vi "RemoteVI Send Frame.vi"(0 "Client":T1, 5 "pixmap":u32[][](array[numeric]), 7 "width":i32, 9 "height":i32, 11 "error in":errorcluster) -> (4 "Client out":T1, 6 "sent?":bool, 15 "error out":errorcluster)   [LabVIEW 2020, in "RemoteVI.lvlib"]
doc: "Sends one FRAME to one client if flow control allows (docs\\protocol.md sections 3.1 and 5). Nothing happens when the client is closed or already has 2 unacknowledged frames (seq - acked >= 2), or when RemoteVI Dirty Rects.vi finds no change against the pixmap this client was last sent. Otherwise every dirty rect is encoded with RemoteVI Encode Rect PNG.vi, the frame is built with RemoteVI Frame Encode.vi (seq + 1, width, height), wrapped in a binary WebSocket frame and written with TCP Write (2 s timeout). On success seq is incremented, last sent becomes pixmap and sent? is TRUE; a write error sets closed instead. error out carries PNG encoding errors."
uses:
  RemoteVI.lvlib
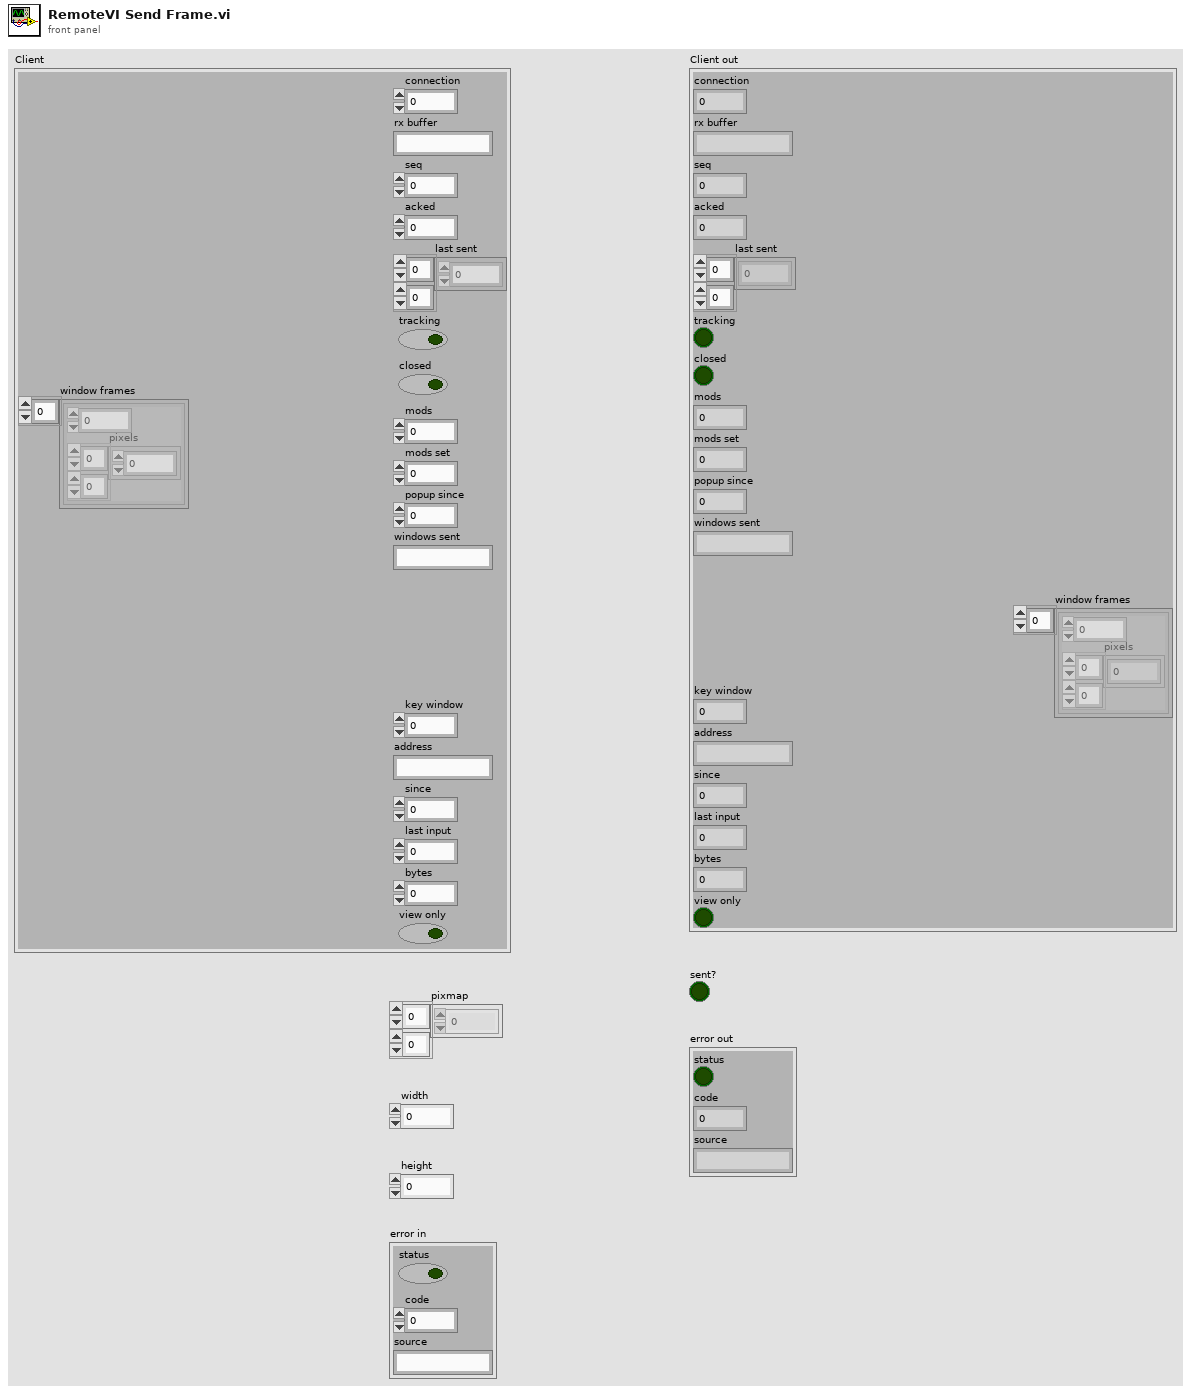
[diagram p1: front panel]
types:
  T1 = cluster{"connection":u32, "rx buffer":string, "seq":u32, "acked":u32, "last sent":u32[][], "tracking":bool, "closed":bool, "mods":u8, "mods set":u8, "popup since":u32, "windows sent":string, "window frames":cluster{"id":u64, "pixels":u32[][]}[], "key window":u64, "address":string, "since":dbl, "last input":dbl, "bytes":dbl, "view only":bool}
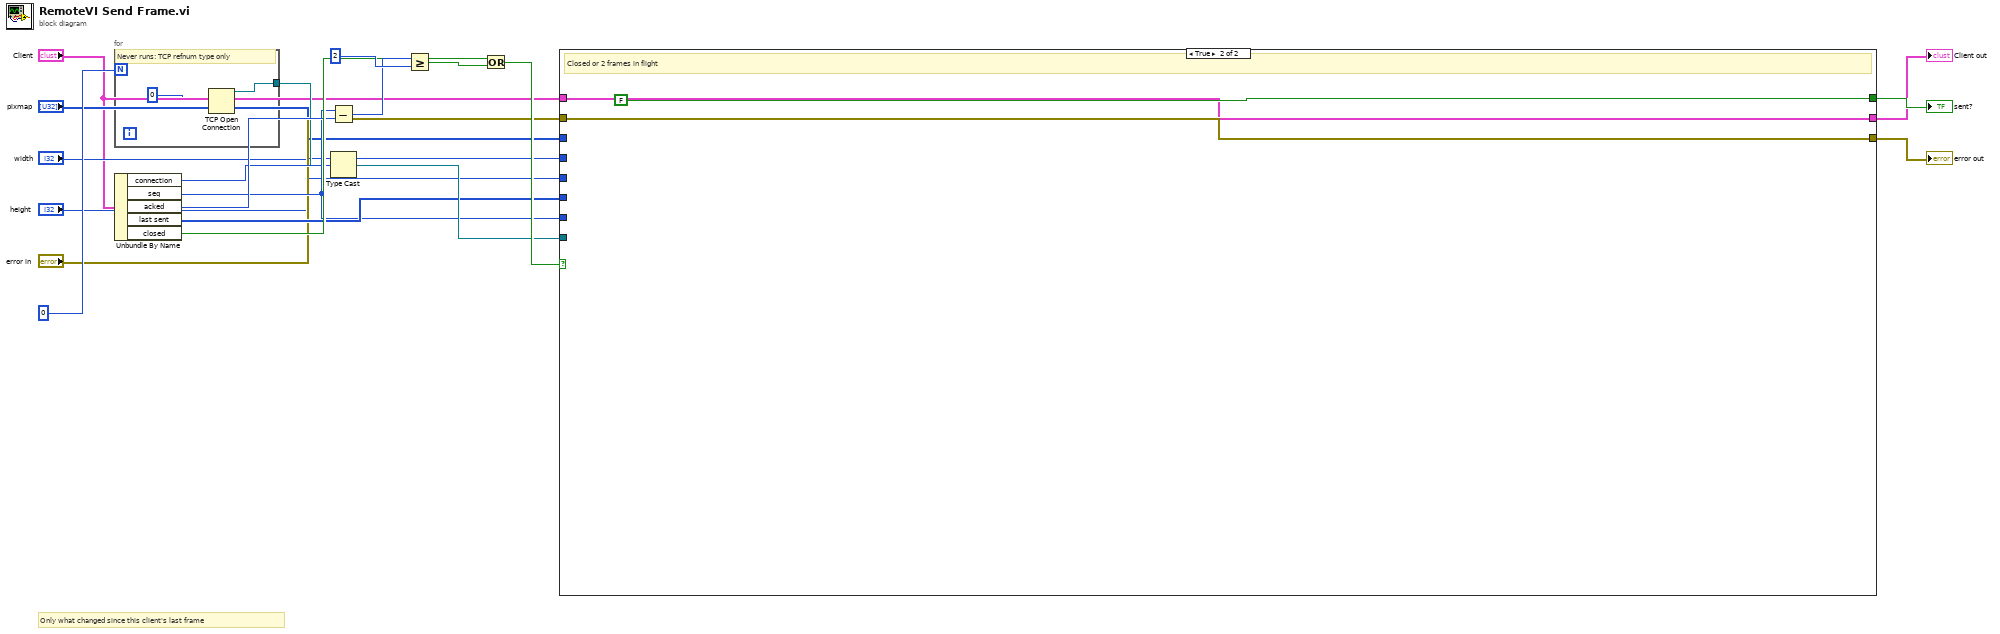
[diagram p0: block diagram]
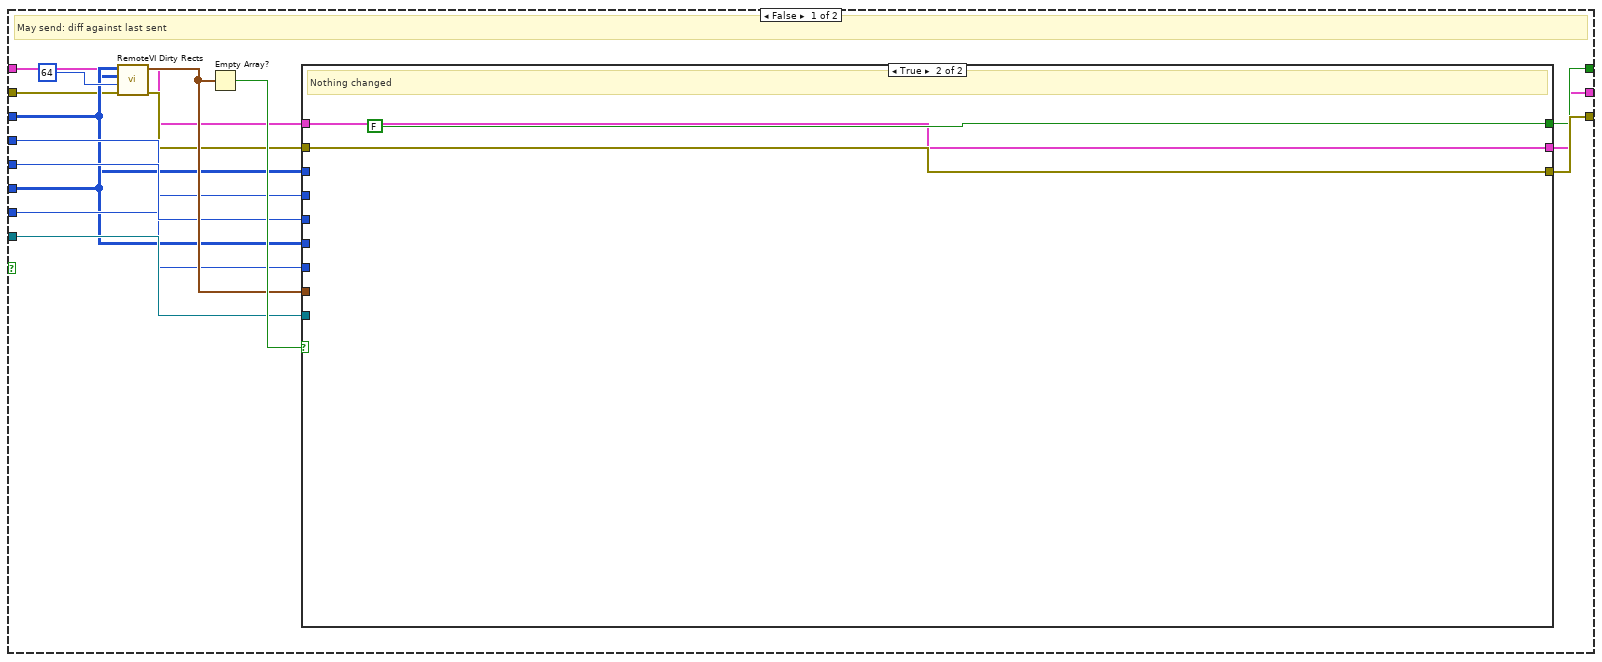
[diagram p2: hidden frame]
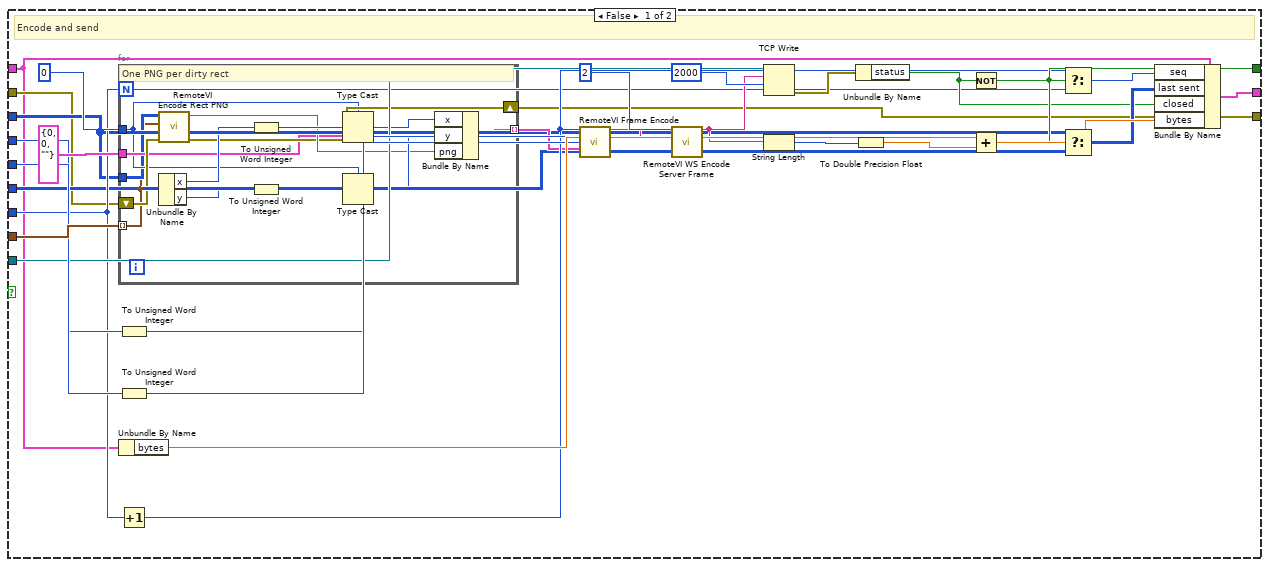
[diagram p3: hidden frame]
diagram:
  # "Only what changed since this client's last frame"
  n1 = for {
    N: 0 -> [_]
    tunnel: [w22] -> w7
    # "Never runs: TCP refnum type only"
    n2 = TCP Open Connection(remote port or service name=u16 0) -> (connection ID=w22:refnum<k5>)  [unwired: 4 in, 1 out]
  }
  n3 = Unbundle By Name("Client") -> ("connection"=w8:u32, "seq"=w9:u32, "acked"=w10:u32, "last sent"=w11:u32[][], "closed"=w12:bool)
  n4 = Subtract(x=w9, y=w10) -> (x-y=w14:u32)
  n5 = Type Cast(type=w7, x=w8) -> (*(type *) &x=w13:refnum<k5>)
  n6 = Greater Or Equal?(x=w14, y=u32 2) -> (x >= y?=w16:bool)
  n7 = Or(x=w12, y=w16) -> (x .or. y?=w17:bool)
  n8 = case shown="True" w17 {
    tunnel: "Client" -> [w23 w84]
    tunnel: "error in" -> [w24 w85]
    tunnel: "pixmap" -> [w25 _]
    tunnel: "width" -> [w29 _]
    tunnel: "height" -> [w30 _]
    tunnel: [w35 FALSE] -> w19
    tunnel: w11 -> [w26 _]
    tunnel: w9 -> [w27 _]
    tunnel: [w34 w84] -> w18
    tunnel: [w36 w85] -> w20
    tunnel: w13 -> [w28 _]
    frame False {
      # "May send: diff against last sent"
      n9 = call "RemoteVI Dirty Rects.vi"("tile size"=64, "current"=w25, "previous"=w26) -> ("rects"=w32:cluster{"x":i32, "y":i32, "w":i32, "h":i32}[])  [unwired: 8 in]
      n10 = Empty Array?(array=w32) -> (empty?=w33:bool)
      n11 = case shown="True" w33 {
        tunnel: [w59 FALSE] -> w35
        tunnel: w23 -> [w37 w81]
        tunnel: w24 -> [w38 w82]
        tunnel: w25 -> [w39 _]
        tunnel: w29 -> [w43 _]
        tunnel: w30 -> [w44 _]
        tunnel: w26 -> [w40 _]
        tunnel: w27 -> [w41 _]
        tunnel: [w66 w81] -> w34
        tunnel: [w48 w82] -> w36
        tunnel: w32 -> [w45 _]
        tunnel: w28 -> [w42 _]
        frame False {
          # "Encode and send"
          n12 = for {
            tunnel: i16 0 -> [w69]
            tunnel: cluster{"x":i16, "y":i16, "png":string} {"x"=0, "y"=0, "png"=""} -> [w70]
            tunnel: w39 -> [w68]
            shift-right: [w72] -> w48
            shift-left: w38 -> [w71]
            tunnel: w45 -> [w67] mode=indexing
            tunnel: [w80] -> w49 mode=indexing
            # "One PNG per dirty rect"
            n13 = call "RemoteVI Encode Rect PNG.vi"("error in"=w71, "rect"=w67, "pixmap"=w68) -> ("error out"=w72:errorcluster, "png"=w73:string)  [unwired: 7 in]
            n14 = Unbundle By Name(w67) -> ("x"=w74:i32, "y"=w75:i32)
            n15 = To Unsigned Word Integer(number=w74) -> (unsigned 16bit integer=w76:u16)
            n16 = To Unsigned Word Integer(number=w75) -> (unsigned 16bit integer=w77:u16)
            n17 = Type Cast(type=w69, x=w76) -> (*(type *) &x=w78:i16)
            n18 = Type Cast(type=w69, x=w77) -> (*(type *) &x=w79:i16)
            n19 = Bundle By Name(cluster=w70, "x"=w78, "y"=w79, "png"=w73) -> (w80:cluster{"x":i16, "y":i16, "png":string})
          }
          n20 = To Unsigned Word Integer(number=w43) -> (unsigned 16bit integer=w51:u16)
          n21 = To Unsigned Word Integer(number=w44) -> (unsigned 16bit integer=w52:u16)
          n22 = Unbundle By Name(w37) -> ("bytes"=w64:dbl)
          n23 = Increment(x=w41) -> (x+1=w50:u32)
          n24 = call "RemoteVI Frame Encode.vi"("seq"=w50, "width"=w51, "height"=w52, "rects"=w49) -> ("message"=w53:string)  [unwired: 11 in]
          n25 = call "RemoteVI WS Encode Server Frame.vi"("opcode"=u8 2, "payload"=w53) -> ("frame"=w55:string)  [unwired: 13 in]
          n26 = TCP Write(connection ID=w42, data in=w55, 9:2000) -> (error out=w57:errorcluster)  [unwired: 1 in, 2 out]
          n27 = String Length(string=w55) -> (length=w62:i32)
          n28 = Unbundle By Name(w57) -> ("status"=w58:bool)
          n29 = To Double Precision Float(number=w62) -> (double precision float=w63:dbl)
          n30 = Not(x=w58) -> (.not. x?=w59:bool)
          n31 = Add(x=w64, y=w63) -> (x+y=w65:dbl)
          n32 = Select(t=w50, s=w59, f=w41) -> (s? t:f=w60:u32)
          n33 = Select(t=w39, s=w59, f=w40) -> (s? t:f=w61:u32[][])
          n34 = Bundle By Name(cluster=w37, "seq"=w60, "last sent"=w61, "closed"=w58, "bytes"=w65) -> (w66:T1)
        }
        frame True {
          # "Nothing changed"
        }
      }
    }
    frame True {
      # "Closed or 2 frames in flight"
    }
  }
  "Client out" <- w18
  "sent?" <- w19
  "error out" <- w20
